vi "Read Relays.vi"(8 "error in (no error)":errorcluster, 11 "Device":string="hidraw0") -> (0 "error out":errorcluster, 3 "Relays":bool[](array[boolean]))   [LabVIEW 2021, in "USB Relay Control.lvlib"]
uses:
  USB Relay Control.lvlib
  typedef/Read Write.ctl
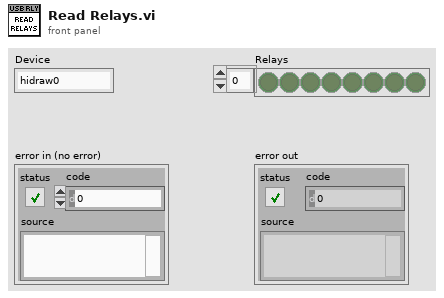
[diagram p1: front panel]
types:
  T1 = typedef "USB Relay Control.lvlib/Read Write.ctl" = enum8{"Read", "Write"}
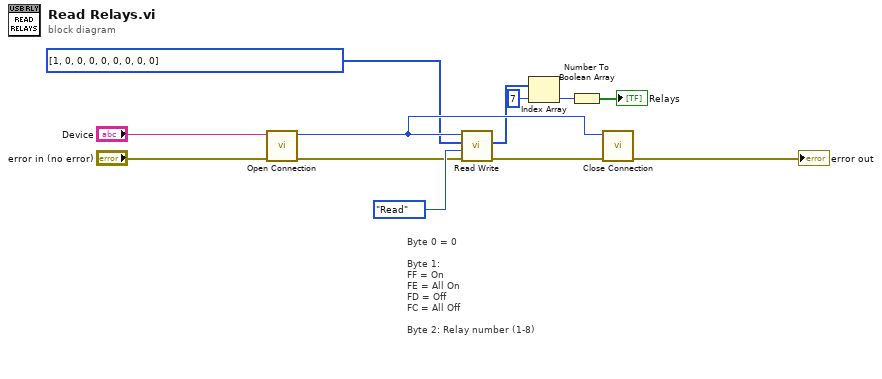
[diagram p0: block diagram]
diagram:
  # "Byte 0 = 0\n\nByte 1:\nFF = On\nFE = All On\nFD = Off\nFC = All Off\n\nByte 2: Relay number (1-8)"
  n1 = call "Open Connection.vi"("error in (no error)"="error in (no error)", "Device"="Device") -> ("error out"=w9:errorcluster, "HID RAW Reference"=w11:i32)  [unwired: 8 in]
  n2 = call "Read Write.vi"("error in (no error)"=w9, "RW"=Read_Write."Read", "Buffer In"=u8[] [1, 0, 0, 0, 0, 0, 0, 0, 0], "HID RAW Reference"=w11) -> ("error out"=w6:errorcluster, "Buffer Out"=w4:u8[])  [unwired: 6 in]
  n3 = Index Array(array=w4, index=7) -> (element=w2:u8)
  n4 = Number To Boolean Array(number=w2) -> (Boolean array=→"Relays":bool[])
  n5 = call "Close Connection.vi"("error in (no error)"=w6, "HID RAW Reference"=w11) -> ("error out"=→"error out":errorcluster)  [unwired: 9 in]
